vi "Initialize.vi"(7 "Time Entry Store in":refnum<class "Time Entry Store-INI.lvclass">, 8 "error in (no error)":errorcluster, 11 "Data Folder":path) -> (0 "error out":errorcluster, 5 "Time Entry Store out":refnum<class "Time Entry Store-INI.lvclass">)   [LabVIEW 2024, in "Time Entry Store-INI.lvclass"]
doc: "Remembers the data folder that holds the month files YYYY-MM.ini. Nothing is read or written here.\n\nGenerated by: Claude"
uses:
  Time Entry Store-INI.lvclass
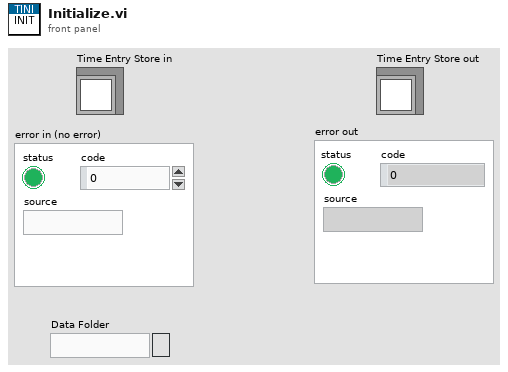
[diagram p1: front panel]
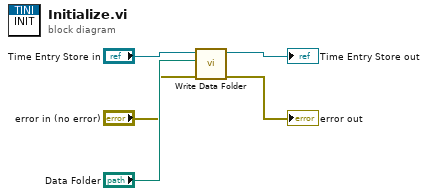
[diagram p0: block diagram]
diagram:
  n1 = call-dynamic "Write Data Folder.vi"("error in (no error)"="error in (no error)", "Data Folder"="Data Folder", "Time Entry Store-INI in"="Time Entry Store in") -> ("error out"=→"error out":errorcluster, "Time Entry Store-INI out"=→"Time Entry Store out":refnum<class "Time Entry Store-INI.lvclass">)  [unwired: 7 in]
